vi "Start Acquisition.vi"(8 "error in (no error)":errorcluster, 11 "ImageHandler:Varex-ImageHandler in":refnum<class "Varex-ImageHandler.lvclass">) -> (0 "error out":errorcluster, 2 "function return":i32, 3 "ImageHandler:Varex-ImageHandler out":refnum<class "Varex-ImageHandler.lvclass">)   [LabVIEW 2022 SP3, in "ImageHandler.lvlib" / "Varex-ImageHandler.lvclass"]
uses:
  Varex-ImageHandler.lvclass
  Varex-ImageHandler.lvclass/Varex-ImageHandler.ctl
  VarexWrapperLvLib/VarexWrapper.lvlib
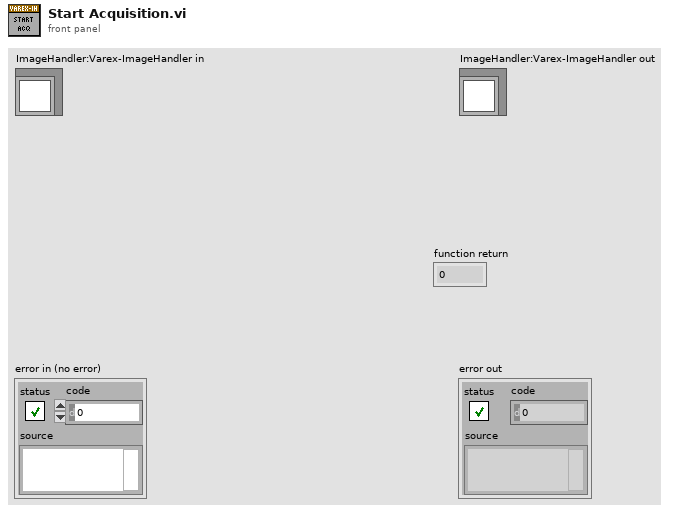
[diagram p1: front panel]
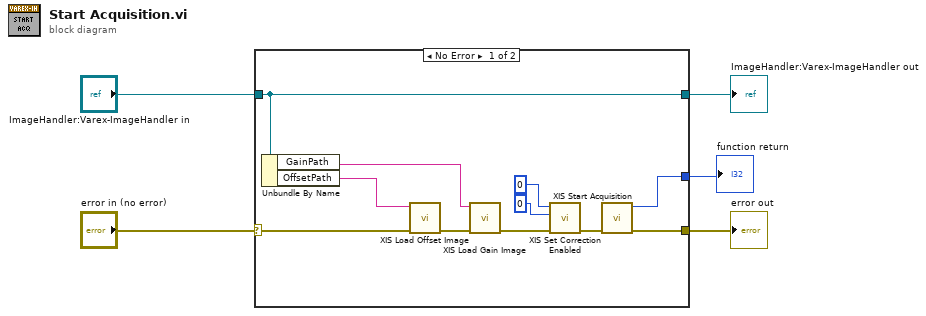
[diagram p0: block diagram]
diagram:
  n1 = case shown="No Error" "error in (no error)" {
    selector: "error in (no error)" -> [w16 w17]
    tunnel: [w15 w17] -> w4
    tunnel: [w8 w18] -> w3
    tunnel: "ImageHandler:Varex-ImageHandler in" -> [w8 w18]
    tunnel: [w9 _] -> w1
    frame No Error {
      n2 = Unbundle By Name(w8) -> ("GainPath"=w6:string, "OffsetPath"=w7:string)
      n3 = call "XIS Load Offset Image.vi"("error in (no error)"=w16, "filePath"=w7) -> ("error out"=w12:errorcluster)  [unwired: 8 in, 1 out]
      n4 = call "XIS Load Gain Image.vi"("error in (no error)"=w12, "filePath"=w6) -> ("error out"=w14:errorcluster)  [unwired: 8 in, 1 out]
      n5 = call "XIS Set Correction Enabled.vi"("error in (no error)"=w14, "enableGain"=0 ("offsetLoaded"), "enableOffset"=0 ("offsetLoaded")) -> ("error out"=w13:errorcluster)  [unwired: 7 in, 1 out]
      n6 = call "XIS Start Acquisition.vi"("error in (no error)"=w13) -> ("error out"=w15:errorcluster, "function return"=w9:i32)  [unwired: 9 in]
    }
    frame Error {
    }
  }
  "error out" <- w4
  "ImageHandler:Varex-ImageHandler out" <- w3
  "function return" <- w1
